vi "Update Value.vi"(6 "Time":dbl, 8 "error in (no error)":errorcluster, 11 "DblPopupControl in":refnum<class "DblPopupControl.lvclass">) -> (0 "error out":errorcluster, 1 "Update":bool, 2 "Value":variant, 3 "DblPopupControl out":refnum<class "DblPopupControl.lvclass">)   [LabVIEW 2020, in "VolatusGUIElements.lvlib" / "DblPopupControl.lvclass"]
uses:
  DblPopupControl.lvclass
  DblPopupControl.lvclass/DblPopupControl.ctl
  lv-vecto/Vecto/Channel DBL/Channel DBL.lvclass/Channel DBL.ctl
  lv-vecto/Vecto/Group DBL/Value by Index.vi
  lv-vecto/Vecto/Channel DBL/Channel DBL.lvclass
  VolatusGUIElements.lvlib
  VolatusGUI/Element Inhibit/Element Inhibit.lvclass
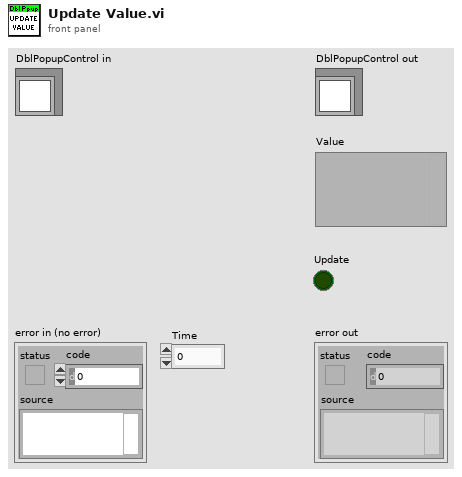
[diagram p1: front panel]
types:
  T1 = typedef "VolatusGUIElements.lvlib/DblPopupControl.lvclass/Cmd State.ctl" = cluster{"Commanding":bool, "Start":dbl, "Error":bool, "Value":dbl}
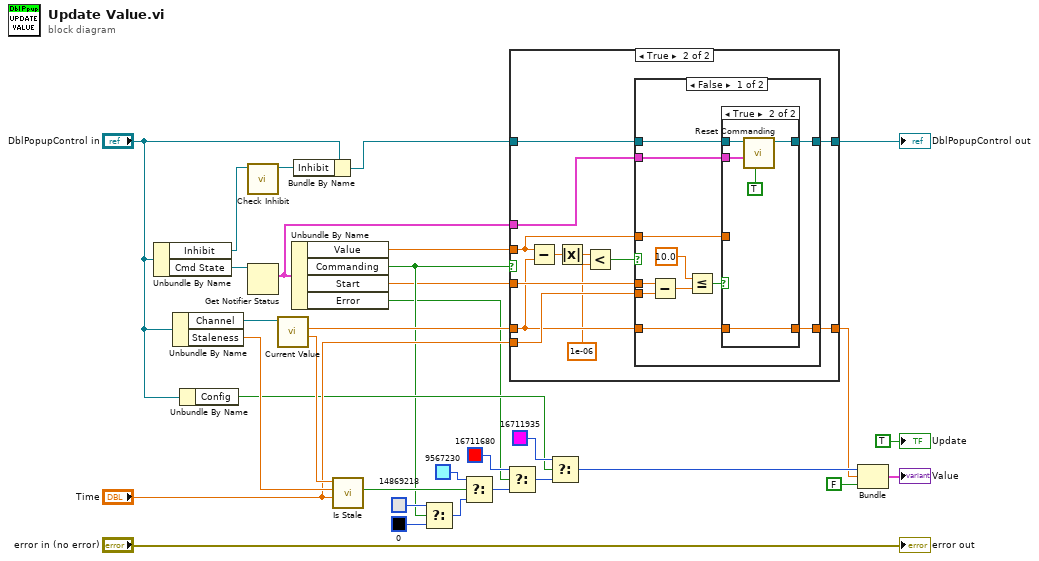
[diagram p0: block diagram]
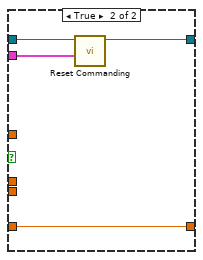
[diagram p4: hidden frame]
diagram:
  n1 = Unbundle By Name("DblPopupControl in") -> ("Inhibit"=w3:refnum<class "Element Inhibit.lvclass">, "Cmd State"=w9:refnum<notifier>)
  n2 = Unbundle By Name("DblPopupControl in") -> ("Channel"=w31:refnum<class "Channel DBL.lvclass">, "Staleness"=w29:dbl)
  n3 = Unbundle By Name("DblPopupControl in") -> ("Config"=w14:bool)
  n4 = call "Check Inhibit.vi"("Element Inhibit in"=w3) -> ("Element Inhibit out"=w1:refnum<class "Element Inhibit.lvclass">)  [unwired: 9 in, 1 out]
  n5 = Get Notifier Status(notifier=w9) -> (current notification=w4:T1)  [unwired: 1 in, 4 out]
  n6 = call "Current Value.vi"("Channel in"=w31) -> ("Timestamp"=w30:dbl, "Scaled"=w19:dbl)  [unwired: 6 in, 3 out]
  n7 = Unbundle By Name(w4) -> ("Value"=w8:dbl, "Commanding"=w7:bool, "Start"=w6:dbl, "Error"=w5:bool)
  n8 = Bundle By Name(cluster="DblPopupControl in", "Inhibit"=w1) -> (w2:refnum<class "DblPopupControl.lvclass">)
  n9 = call "Is Stale.vi"("Time"="Time", "Staleness"=w29, "Timestamp"=w30) -> ("Stale"=w23:bool)  [unwired: 8 in]
  n10 = Select(t=u32 14869218, s=w7, f=u32 0) -> (s? t:f=w13:u32)
  n11 = Select(t=u32 9567230, s=w23, f=w13) -> (s? t:f=w27:u32)
  n12 = Select(t=u32 16711680, s=w5, f=w27) -> (s? t:f=w25:u32)
  n13 = case shown="True" w7 {
    tunnel: w19 -> [w34 w44]
    tunnel: w6 -> [_ w46]
    tunnel: "Time" -> [_ w45]
    tunnel: w8 -> [_ w40]
    tunnel: w2 -> [w33 w43]
    tunnel: [w33 w42] -> w17
    tunnel: [w34 w41] -> w16
    tunnel: w4 -> [_ w35]
    frame False {
    }
    frame True {
      n14 = Subtract(x=w40, y=w44) -> (x-y=w39:dbl)
      n15 = Absolute Value(x=w39) -> (abs(x)=w38:dbl)
      n16 = Less?(x=w38, y=1e-06) -> (x < y?=w36:bool)
      n17 = case shown="False" w36 {
        tunnel: w46 -> [w57 _]
        tunnel: w45 -> [w56 _]
        tunnel: w44 -> [w50 w67]
        tunnel: w43 -> [w52 w68]
        tunnel: [w51 w66] -> w42
        tunnel: [w48 w67] -> w41
        tunnel: w40 -> [w49 _]
        tunnel: w35 -> [w47 w65]
        frame False {
          n18 = Subtract(x=w57, y=w56) -> (x-y=w55:dbl)
          n19 = Less Or Equal?(x=10.0, y=w55) -> (x <= y?=w53:bool)
          n20 = case shown="True" w53 {
            tunnel: w52 -> [w58 w63]
            tunnel: [w58 w62] -> w51
            tunnel: w50 -> [_ w64]
            tunnel: w49 -> [w59 _]
            tunnel: [w59 w64] -> w48
            tunnel: w47 -> [_ w61]
            frame False {
            }
            frame True {
              n21 = call "Reset Commanding.vi"("Error (F)"=TRUE, "Cmd State"=w61, "DblPopupControl in"=w63) -> ("DblPopupControl out"=w62:refnum<class "DblPopupControl.lvclass">)  [unwired: 7 in, 1 out]
            }
          }
        }
        frame True {
          n22 = call "Reset Commanding.vi"("Cmd State"=w65, "DblPopupControl in"=w68) -> ("DblPopupControl out"=w66:refnum<class "DblPopupControl.lvclass">)  [unwired: 8 in, 1 out]
        }
      }
    }
  }
  "DblPopupControl out" <- w17
  n23 = Select(t=u32 16711935, s=w14, f=w25) -> (s? t:f=w22:u32)
  n24 = Bundle(w22, "Scaled"=w16, FALSE) -> (→"Value":cluster{u32, "Scaled":dbl, bool})  [unwired: 1 in]
  "error out" <- "error in (no error)"
  "Update" <- TRUE ("Update")
